vi "wiringPiI2CSetup.vi"(8 "error in (no error)":errorcluster, 11 "devID":i32) -> (0 "error out":errorcluster, 3 "return":T1)   [LabVIEW 2020, in "wiringPi.lvlib"]
doc: "<b>_______________________________________________________________</b>\n** Author: Juan José Villacorta\n** LabVIEW wrapper for C library <b> wiringPi </b>,\n** https://github.com/WiringPi/WiringPi\n<b>_______________________________________________________________</b>\n\n/*\n * wiringPiI2CSetup:\n * Open the I2C device, and regsiter the target device\n *********************************************************************************\n */"
uses:
  wiringPi.lvlib
  Type Defs/I2C Device.ctl
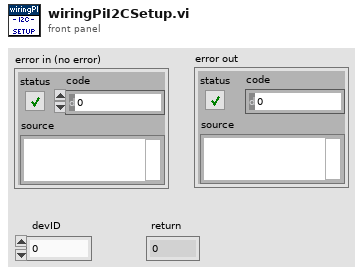
[diagram p1: front panel]
types:
  T1 = typedef "wiringPi.lvlib/I2C Device.ctl" = i32
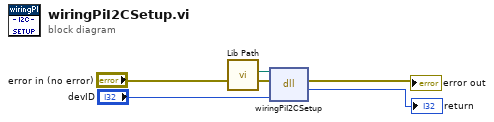
[diagram p0: block diagram]
diagram:
  n1 = call "Lib Path.vi"() -> ("path out"=w2:path)  [unwired: 11 in]
  n2 = dll-call lib="libLVwiringPI.so" fn="wiringPiI2CSetup"(path in=w2, error in="error in (no error)", "devId"="devID") -> (error out=→"error out":errorcluster, "return type"=→"return":i32)  [unwired: 2 in, 1 out]
